vi "DUT Bring Up Pin & Pattern.vi"(11 ".dutbringup File Path":path) -> (1 "Bring-up Pattern":string, 2 "Post Source Delay":dbl[](array[numeric]) format="%#_6p", 3 "Power Sequence Pins":string[](array[string]))   [LabVIEW 2025, in "Digital Pattern Sequencer.lvclass"]
uses:
  Digital Pattern Sequencer.lvclass
  Digital Pattern Sequencer.lvclass/Digital Pattern Sequencer.ctl
  <resource>/objmgr/DOMUserDefRef.rc
  <vilib>/xml/NI_XML.lvlib
  <vilib>/xml/XPath/Get All Matched Nodes (String).vi
  <vilib>/xml/Load XML String.vi
  <vilib>/xml/XPath/Get First Matched Node (String).vi
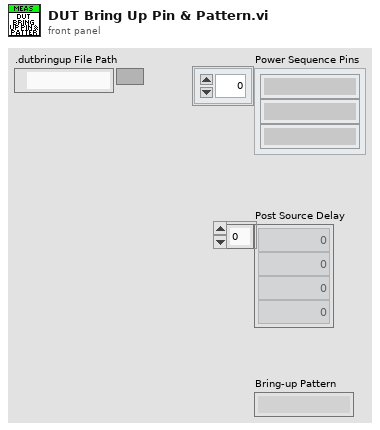
[diagram p1: front panel]
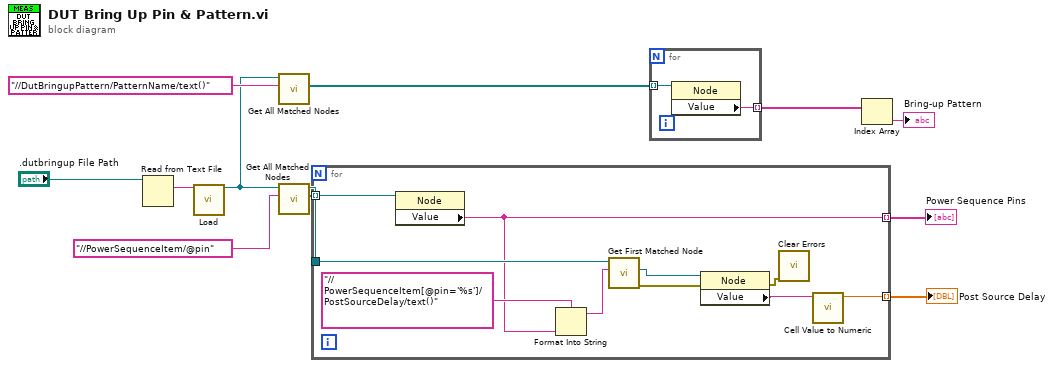
[diagram p0: block diagram]
diagram:
  n1 = Read from Text File(file (use dialog)=".dutbringup File Path") -> (text=w11:string)  [unwired: 3 in, 3 out]
  n2 = call-poly <vilib>:"Load.vi"("XML string"=w11) -> ("DOM document out"=w4:refnum<k20>)  [unwired: 12 in, 2 out]
  n3 = call-poly <vilib>:"Get All Matched Nodes.vi"("XPath expression"="//DutBringupPattern/PatternName/text()", "node in"=w4) -> ("node result array"=w7:refnum<k20>[])  [unwired: 7 in, 2 out]
  n4 = call-poly <vilib>:"Get All Matched Nodes.vi"("XPath expression"="//PowerSequenceItem/@pin", "node in"=w4) -> ("node result array"=w12:refnum<k20>[], "node out"=w3:refnum<k20>)  [unwired: 7 in, 1 out]
  n5 = for {
    tunnel: w12 -> [w22] mode=indexing
    tunnel: [w18] -> w10 mode=indexing
    tunnel: w3 -> [w20]
    tunnel: [w13] -> w2 mode=indexing
    n6 = property class="Node"(reference=w22) -> ("Value"=w18:string)  [unwired: 1 in, 2 out]
    n7 = Format Into String(format string="//PowerSequenceItem[@pin='%s']/PostSourceDelay/text()" ("XPath expression"), w18) -> (resulting string=w17:string)  [unwired: 2 in, 1 out]
    n8 = call-poly <vilib>:"Get First Matched Node.vi"("XPath expression"=w17, "node in"=w20) -> ("error out"=w15:errorcluster, "node result"=w21:refnum<k20>)  [unwired: 7 in, 1 out]
    n9 = property class="Node"(reference=w21, error in=w15) -> (error out=w14:errorcluster, "Value"=w16:string)  [unwired: 1 out]
    n10 = call <vilib>:"Clear Errors.vi"("error in (no error)"=w14) -> ()  [unwired: 5 in, 2 out]
    n11 = call "Cell Value to Numeric.vi"("Cell Value"=w16) -> ("Numeric"=w13:dbl)  [unwired: 9 in, 1 out]
  }
  "Power Sequence Pins" <- w10
  "Post Source Delay" <- w2
  n12 = for {
    tunnel: w7 -> [w24] mode=indexing
    tunnel: [w23] -> w5 mode=indexing
    n13 = property class="Node"(reference=w24) -> ("Value"=w23:string)  [unwired: 1 in, 2 out]
  }
  n14 = Index Array(array=w5) -> (element=→"Bring-up Pattern":string)  [unwired: 1 in]
